vi "Get StationGlobal.vi"() -> ()   [LabVIEW 2020]
uses:
  Engine/Get StationGlobals Prop.vi
  VariableContainer/VariableContainer.lvclass
  Engine/Engine.lvclass
panel:
  out "error out":errorcluster
  out "Original Value":string
  in  "Lookup String":string="Channel"
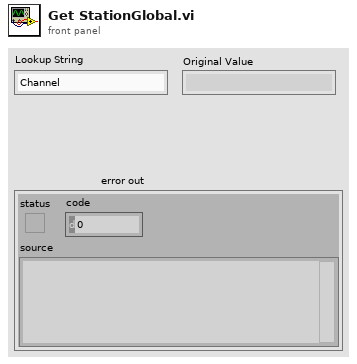
[diagram p1: front panel]
types:
  T1 = typedef "TSS.lvlib/Engine.lvclass/Session Handle.ctl" = refnum<data-value>
  T2 = typedef "TSS.lvlib/VariableContainer.lvclass/Session Handle.ctl" = refnum<data-value>
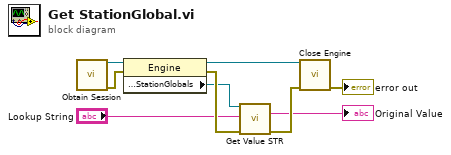
[diagram p0: block diagram]
diagram:
  n1 = call "Obtain Session.vi"() -> ("Session Handle"=w5:T1, "error out"=w7:errorcluster)  [unwired: 14 in]
  n2 = property class="Engine"(reference=w5, error in=w7) -> (reference out=w2:T1, error out=w6:errorcluster, "Properties:StationGlobals"=w4:T2)
  n3 = call "Get Value STR.vi"("Session Handle in"=w4, "Lookup String"="Lookup String", "error in (no error)"=w6) -> ("Value"=→"Original Value":string, "error out"=w9:errorcluster)  [unwired: 9 in, 2 out]
  n4 = call "Close Engine.vi"("Session Handle in"=w2, "error in (no error)"=w9) -> ("error out"=→"error out":errorcluster)  [unwired: 13 in]
